vi "GDSAPI_AddDesignPattern.vi"(8 "error in (no error)":errorcluster, 10 "InterfaceClass(*.lvclass)":path, 11 "ClassPath(*.lvclass)":path) -> (0 "error out":errorcluster)   [LabVIEW 2020]
doc: "This VI creates Methods in a class."
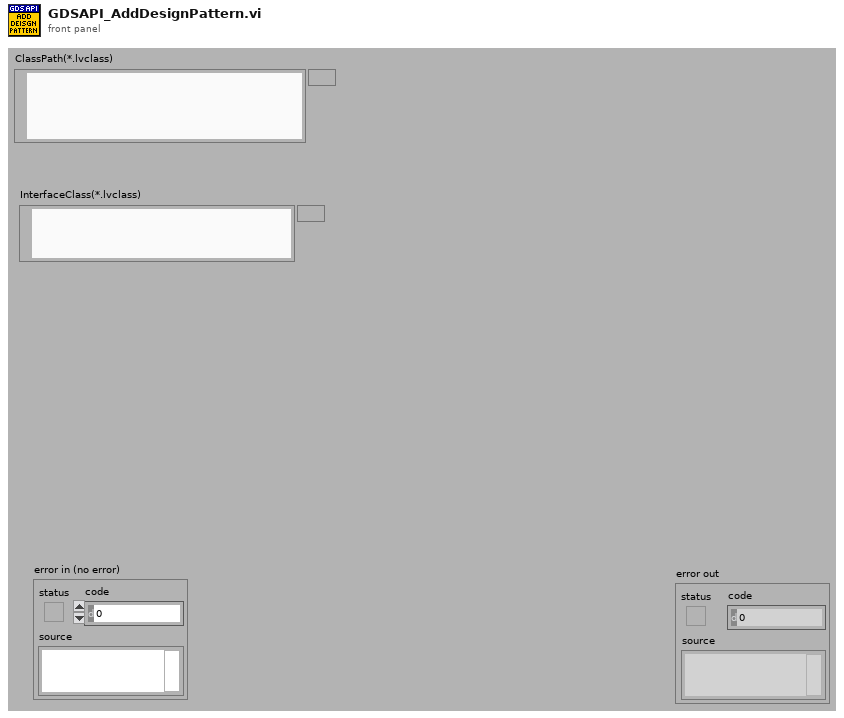
[diagram p1: front panel]
types:
  T1 = typedef "GDSLvCLass_ClassSettingsType.ctl" = cluster{"ClassProviderName":string, "ClassTemplateUsed":string, "ClassTemplateVersion":string, "ClassDescription":string, "PlugIns":T2[], "ConnectorPanePattern":string}
  T2 = typedef "GDSLvClass_PlugIn.ctl" = cluster{"Type":T3, "ID":string, "Version":string, "Path":path, "Name":string, "Data":variant}
  T3 = typedef "GDSLvClass_PlugInTypes.ctl" = enum16{"DesignPattern", "MethodTypes"}
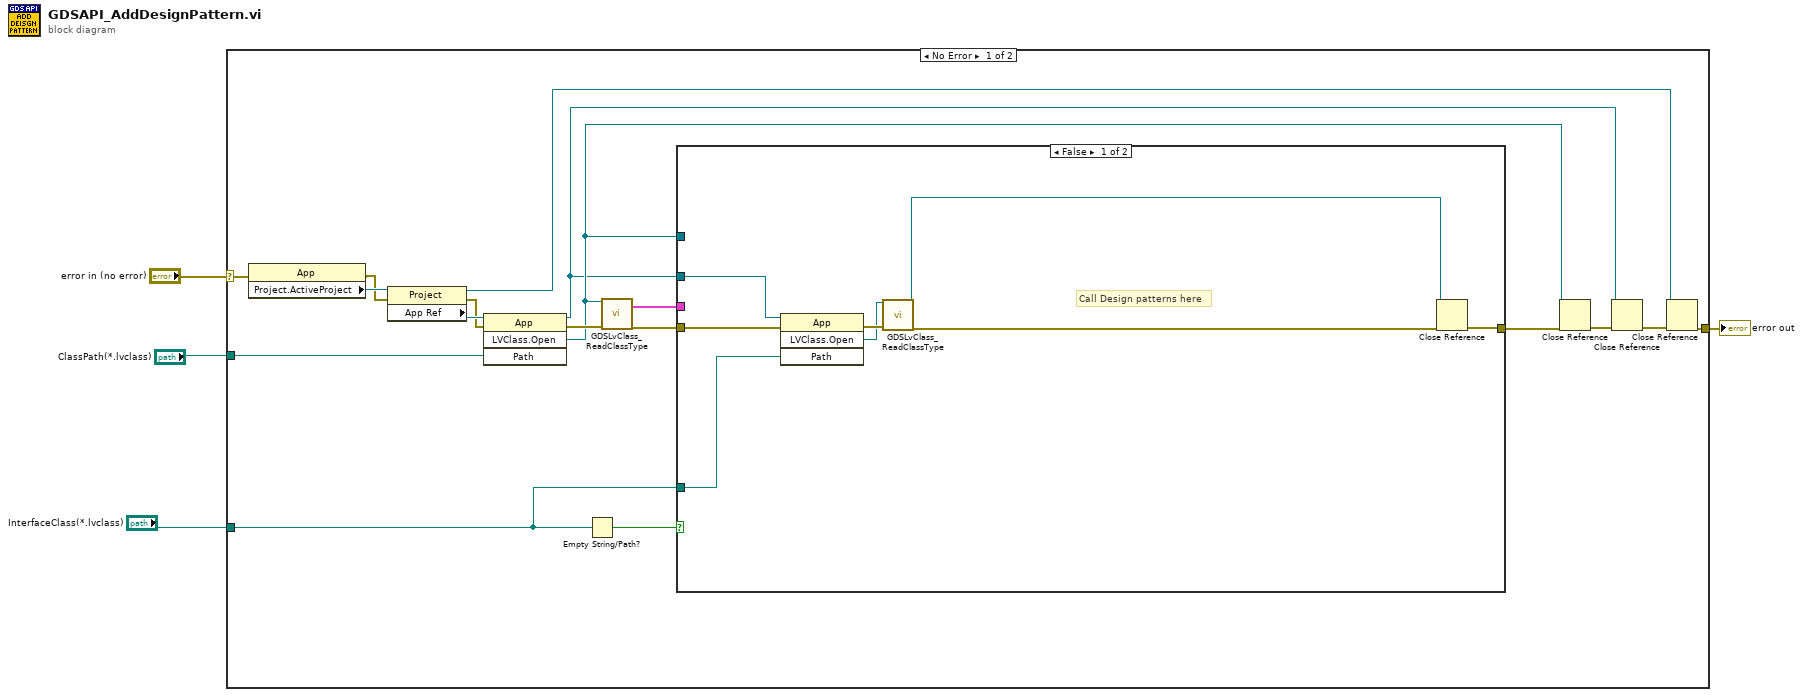
[diagram p0: block diagram]
diagram:
  n1 = case shown="No Error" "error in (no error)" {
    selector: "error in (no error)" -> [w5 w32]
    tunnel: "ClassPath(*.lvclass)" -> [w22 _]
    tunnel: [w15 w32] -> w3
    tunnel: "InterfaceClass(*.lvclass)" -> [w8 _]
    frame No Error {
      n2 = property class="App"(error in=w5) -> (error out=w18:errorcluster, "Project.ActiveProject"=w21:refnum<vi>)  [unwired: 1 in, 1 out]
      n3 = property class="Project"(reference=w21, error in=w18) -> (reference out=w11:refnum<vi>, error out=w19:errorcluster, "App Ref"=w20:refnum<vi>)
      n4 = invoke class="App" method="LVClass.Open"(reference=w20, error in=w19, "Path"=w22) -> (reference out=w6:refnum<vi>, error out=w14:errorcluster, "LVClass.Open"=w10:refnum<vi>)  [unwired: 1 in, 1 out]
      n5 = Empty String/Path?(string/path=w8) -> (empty?=w9:bool)
      n6 = call "GDSLvClass_ReadClassType.vi"("Class Refnum In"=w10, "error in (no error)"=w14) -> ("ClassSettings"=w12:T1, "error out"=w13:errorcluster)  [unwired: 15 in, 1 out]
      n7 = case shown="False" w9 {
        tunnel: w13 -> [w30 w31]
        tunnel: w12 -> [_ _]
        tunnel: w10 -> [_ _]
        tunnel: w8 -> [w26 _]
        tunnel: [w25 w31] -> w7
        tunnel: w6 -> [w29 _]
        frame False {
          # "Call Design patterns here"
          n8 = invoke class="App" method="LVClass.Open"(reference=w29, error in=w30, "Path"=w26) -> (error out=w28:errorcluster, "LVClass.Open"=w27:refnum<vi>)  [unwired: 1 in, 2 out]
          n9 = call "GDSLvClass_ReadClassType.vi"("Class Refnum In"=w27, "error in (no error)"=w28) -> ("Class Refnum Out"=w24:refnum<vi>, "error out"=w23:errorcluster)  [unwired: 15 in, 1 out]
          n10 = Close Reference(reference=w24, error in (no error)=w23) -> (error out=w25:errorcluster)
        }
        frame True {
        }
      }
      n11 = Close Reference(reference=w10, error in (no error)=w7) -> (error out=w17:errorcluster)
      n12 = Close Reference(reference=w6, error in (no error)=w17) -> (error out=w16:errorcluster)
      n13 = Close Reference(reference=w11, error in (no error)=w16) -> (error out=w15:errorcluster)
    }
    frame Error {
    }
  }
  "error out" <- w3
